vi "SA mark MAX Peak.vi"(8 "error in (no error)":errorcluster caption="에러 입력(에러 없음)", 11 "Instrument Manager 입력":refnum<class "Instrument Manager.lvclass">) -> (0 "error out":errorcluster caption="에러 출력", 3 "Instrument Manager 출력":refnum<class "Instrument Manager.lvclass">)   [LabVIEW 2023, in "Instrument Manager.lvclass"]
uses:
  Instrument Manager.lvclass
  Module/Spectrum Analyzer/TYPE DEFINITION/TYPE Marker Control Mode.ctl
  Module/Spectrum Analyzer/TYPE DEFINITION/TYPE Marker Peak Search Type.ctl
  Instrument Manager.lvclass/Instrument Manager.ctl
  Module/Spectrum Analyzer/Interface_Spectrum/Interface_Spectrum.lvclass
  Module/Spectrum Analyzer/Spectrum Analyzer.lvlib
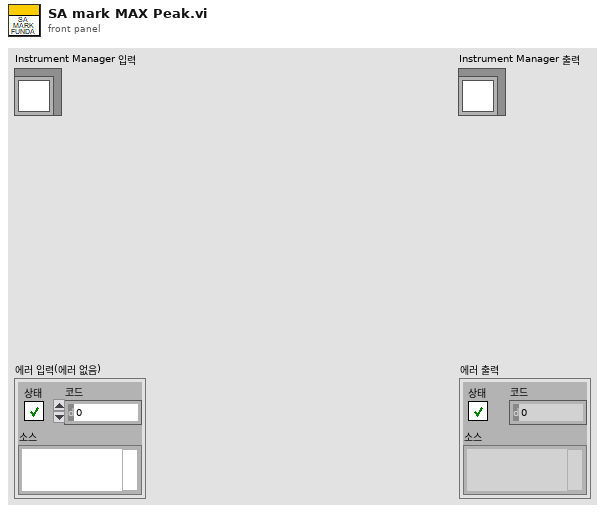
[diagram p1: front panel]
types:
  T1 = typedef "Spectrum Analyzer.lvlib/TYPE Marker Peak Search Type.ctl" = enum16{"Max", "Next Peak", "Max - Auto"}
  T2 = typedef "Spectrum Analyzer.lvlib/TYPE Marker Control Mode.ctl" = enum16{"Normal", "Delta", "Off"}
  T3 = cluster{"Anritsu Call Box":refnum<class "Anritsu Call Box.lvclass">, "Spectrum Analyzer":refnum<class "Interface_Spectrum.lvclass">, "RF Switch Box":refnum<class "RF Filter Box.lvclass">, "Turn Table":refnum<class "Interface - Turn Table.lvclass">, "Mast":refnum<class "Interface - Mast.lvclass">, "3D Controller":refnum<class "Interface_3D Controller.lvclass">}
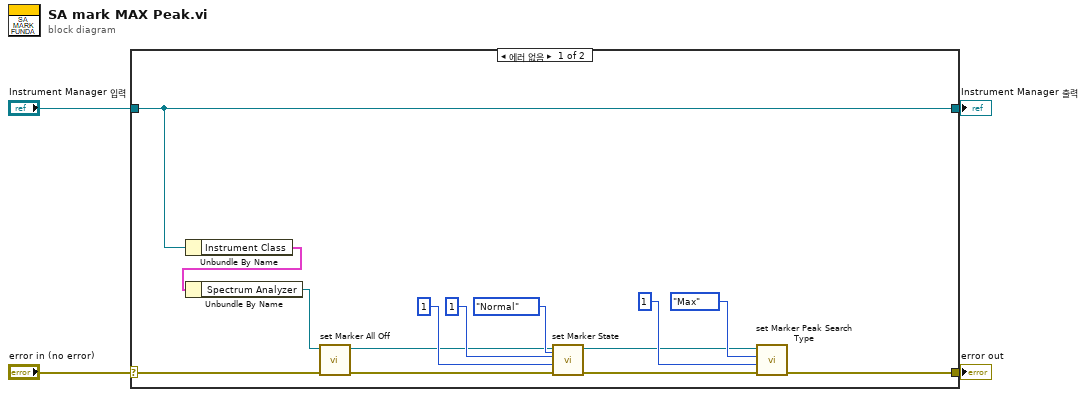
[diagram p0: block diagram]
diagram:
  n1 = case shown="에러 없음" "error in (no error)" {
    selector: "error in (no error)" -> [w7 w20]
    tunnel: [w6 w20] -> w3
    tunnel: [w9 w19] -> w1
    tunnel: "Instrument Manager 입력" -> [w9 w19]
    frame No Error {
      n2 = Unbundle By Name(w9) -> ("Instrument Class"=w8:T3)
      n3 = Unbundle By Name(w8) -> ("Spectrum Analyzer"=w5:refnum<class "Interface_Spectrum.lvclass">)
      n4 = call-dynamic "set Marker All Off.vi"("error in (no error)"=w7, "Interface_Spectrum in"=w5) -> ("error out"=w10:errorcluster, "Interface_Spectrum out"=w15:refnum<class "Interface_Spectrum.lvclass">)  [unwired: 8 in]
      n5 = call-dynamic "set Marker State.vi"("Marker Mode"=TYPE_Marker_Control_Mode."Normal", "error in (no error)"=w10, "trace index"=1, "Marker Index"=1, "Interface_Spectrum in"=w15) -> ("error out"=w11:errorcluster, "Interface_Spectrum out"=w12:refnum<class "Interface_Spectrum.lvclass">)  [unwired: 5 in]
      n6 = call-dynamic "set Marker Peak Search Type.vi"("error in (no error)"=w11, "Marker Index"=1, "Peak Search Type"=TYPE_Marker_Peak_Search_Type."Max", "Interface_Spectrum in"=w12) -> ("error out"=w6:errorcluster)  [unwired: 6 in, 1 out]
    }
    frame Error {
    }
  }
  "error out" <- w3
  "Instrument Manager 출력" <- w1
